vi "VIH Project Tree - Add Files - Build Item Tags.vi"(11 "Items Array":T2[](array[typedef])) -> (2 "Item Items Data":T1(array[cluster]), 3 "Item Parent Tags":string[](array[string]))   [LabVIEW 2014]
doc: "::: VI Helpeks :::\nCopyright (c) 2000-2026 Konstantin Shifershteyn. All rights reserved."
uses:
  _VIH HelpGen - Palette.llb/VIH HelpGen Typedef - Palette - Item Info Cluster.ctl
  _VIH HelpGen - Palette.llb/VIH HelpGen Typedef - Palette - Item Type Enum.ctl
  VIH Project Tree Typedef - Tree Item Type.ctl
panel:
  # "VI Helpeks\nCopyright (c) 2012-2026 Konstantin Shifershteyn"
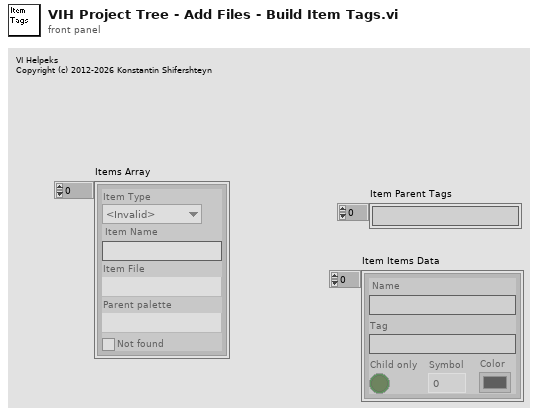
[diagram p1: front panel]
types:
  T1 = cluster{"Name":string, "Tag":string, "Child only":bool, "Symbol":i32, "Color":u32}[]
  T2 = typedef "VIH HelpGen Typedef - Palette - Item Info Cluster.ctl" = cluster{"Item Type":T3, "Item Name":string, "Item File":path, "Parent palette":path, "Not found":bool}
  T3 = typedef "VIH HelpGen Typedef - Palette - Item Type Enum.ctl" = enum32{"<Invalid>", "<unknown>", "VI", "Menu", "LV Func", "Express VI", "Poly VI", "CTL", "HTML"}
  T4 = cluster{"Name":string, "Tag":string, "Child only":bool, "Symbol":i32, "Color":u32}
  T5 = typedef "VIH Project Tree Typedef - Tree Item Type.ctl" = enum32{"<Invalid>", "Project", "Proj Files", "Proj Rules", "File Group", "Rule Group", "Any File", "LV Func", ".mnu", ".mnu (dyn)", ".vi", ".vi (dyn)", ".vit", ".vit (dyn)", ".ctl", ".ctl (dyn)", ".ctt", ".ctt (dyn)", "polyVI", "polyVI (dyn)", "expVI", "expVI (dyn)", "HTML", "PolyVI Inst"}
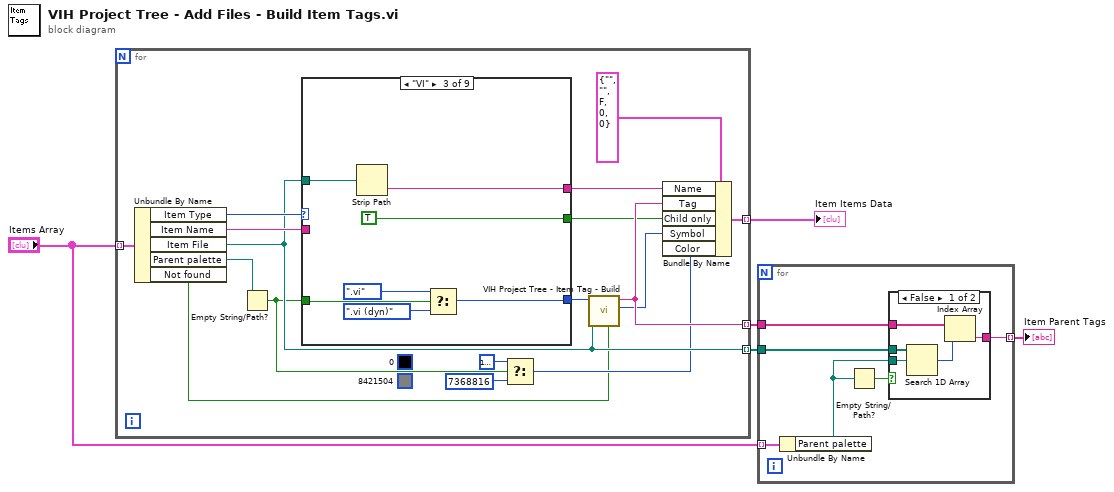
[diagram p0: block diagram]
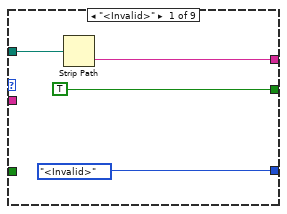
[diagram p3: hidden frame]
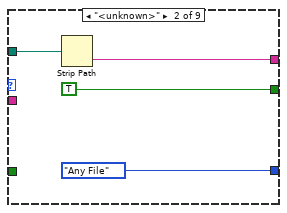
[diagram p4: hidden frame]
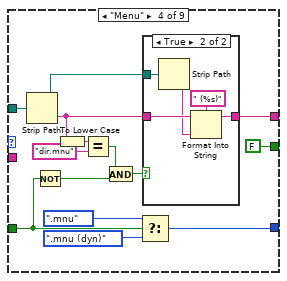
[diagram p5: hidden frame]
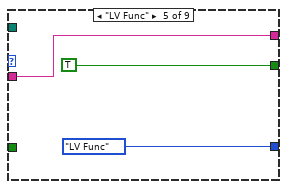
[diagram p7: hidden frame]
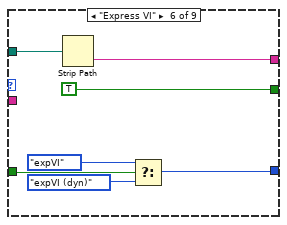
[diagram p8: hidden frame]
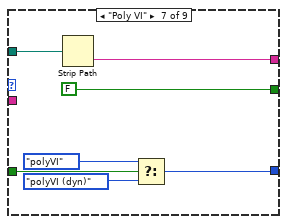
[diagram p9: hidden frame]
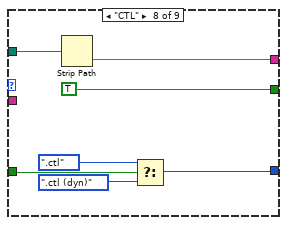
[diagram p10: hidden frame]
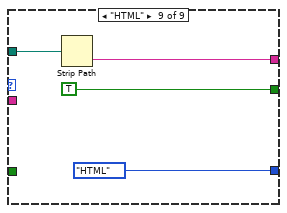
[diagram p11: hidden frame]
diagram:
  n1 = for {
    tunnel: "Items Array" -> [w22] mode=indexing
    tunnel: [w14] -> w3 mode=indexing
    tunnel: [w19] -> w4 mode=indexing
    tunnel: [w11] -> w1 mode=indexing
    (unwired) u32 8421504
    (unwired) u32 0
    n2 = Unbundle By Name(w22) -> ("Item Type"=w21:T3, "Item Name"=w20:string, "Item File"=w19:path, "Parent palette"=w18:path, "Not found"=w6:bool)
    n3 = Empty String/Path?(string/path=w18) -> (empty?=w10:bool)
    n4 = case shown="\"VI\"" w21 {
      tunnel: [TRUE TRUE TRUE FALSE TRUE TRUE FALSE TRUE TRUE] -> w12
      tunnel: w10 -> [_ _ w33 w44 _ w63 w70 w77 _]
      tunnel: [VIH_Project_Tree_Typedef_-_Tree_Item_Type."<Invalid>" ("Item Type") VIH_Project_Tree_Typedef_-_Tree_Item_Type."Any File" ("Item Type") w34 w48 VIH_Project_Tree_Typedef_-_Tree_Item_Type."LV Func" ("Item Type") w64 w71 w78 VIH_Project_Tree_Typedef_-_Tree_Item_Type."HTML" ("Item Type")] -> w17
      tunnel: w20 -> [_ _ _ _ w58 _ _ _ _]
      tunnel: [w23 w28 w31 w40 w58 w61 w68 w75 w83] -> w15
      tunnel: w19 -> [w24 w29 w32 w47 _ w62 w69 w76 w84]
      frame "<Invalid>" {
        n5 = Strip Path(path=w24) -> (name=w23:string)  [unwired: 1 out]
      }
      frame "<unknown>" {
        n6 = Strip Path(path=w29) -> (name=w28:string)  [unwired: 1 out]
      }
      frame "VI" {
        n7 = Strip Path(path=w32) -> (name=w31:string)  [unwired: 1 out]
        n8 = Select(t=VIH_Project_Tree_Typedef_-_Tree_Item_Type.".vi" ("Item Type"), s=w33, f=VIH_Project_Tree_Typedef_-_Tree_Item_Type.".vi (dyn)" ("Item Type")) -> (s? t:f=w34:T5)
      }
      frame "Menu" {
        n9 = Strip Path(path=w47) -> (stripped path=w38:path, name=w39:string)
        n10 = Not(x=w44) -> (.not. x?=w43:bool)
        n11 = To Lower Case(string=w39) -> (all lower case string=w46:string)
        n12 = Equal?(x=w46, y="dir.mnu") -> (x = y?=w42:bool)
        n13 = And(x=w42, y=w43) -> (x .and. y?=w41:bool)
        n14 = Select(t=VIH_Project_Tree_Typedef_-_Tree_Item_Type.".mnu" ("Item Type"), s=w44, f=VIH_Project_Tree_Typedef_-_Tree_Item_Type.".mnu (dyn)" ("Item Type")) -> (s? t:f=w48:T5)
        n15 = case shown="True" w41 {
          tunnel: [w52 w55] -> w40
          tunnel: w39 -> [w52 w56]
          tunnel: w38 -> [_ w57]
          frame False {
          }
          frame True {
            n16 = Strip Path(path=w57) -> (name=w54:string)  [unwired: 1 out]
            n17 = Format Into String(format string=" (%s)", initial string=w56, w54) -> (resulting string=w55:string)  [unwired: 1 in, 1 out]
          }
        }
      }
      frame "LV Func" {
      }
      frame "Express VI" {
        n18 = Strip Path(path=w62) -> (name=w61:string)  [unwired: 1 out]
        n19 = Select(t=VIH_Project_Tree_Typedef_-_Tree_Item_Type."expVI" ("Item Type"), s=w63, f=VIH_Project_Tree_Typedef_-_Tree_Item_Type."expVI (dyn)" ("Item Type")) -> (s? t:f=w64:T5)
      }
      frame "Poly VI" {
        n20 = Strip Path(path=w69) -> (name=w68:string)  [unwired: 1 out]
        n21 = Select(t=VIH_Project_Tree_Typedef_-_Tree_Item_Type."polyVI" ("Item Type"), s=w70, f=VIH_Project_Tree_Typedef_-_Tree_Item_Type."polyVI (dyn)" ("Item Type")) -> (s? t:f=w71:T5)
      }
      frame "CTL" {
        n22 = Strip Path(path=w76) -> (name=w75:string)  [unwired: 1 out]
        n23 = Select(t=VIH_Project_Tree_Typedef_-_Tree_Item_Type.".ctl" ("Item Type"), s=w77, f=VIH_Project_Tree_Typedef_-_Tree_Item_Type.".ctl (dyn)" ("Item Type")) -> (s? t:f=w78:T5)
      }
      frame "HTML" {
        n24 = Strip Path(path=w84) -> (name=w83:string)  [unwired: 1 out]
      }
    }
    n25 = Select(t=u32 16777228, s=w10, f=u32 7368816) -> (s? t:f=w8:u32)
    n26 = call "VIH Project Tree - Item Tag - Build.vi"("Not found"=w6, "Item File Path"=w19, "Item Type"=w17) -> ("Tree Item Symbol"=w13:i32, "Tree Item Tag"=w14:string)  [unwired: 7 in]
    n27 = Bundle By Name(cluster=T4 {"Name"="", "Tag"="", "Child only"=FALSE, "Symbol"=0, "Color"=0} ("Tree Item Data"), "Name"=w15, "Tag"=w14, "Child only"=w12, "Symbol"=w13, "Color"=w8) -> (w11:T4)
  }
  "Item Items Data" <- w1
  n28 = for {
    tunnel: "Items Array" -> [w91] mode=indexing
    tunnel: w4 -> [w90]
    tunnel: w3 -> [w89]
    tunnel: [w88] -> w2 mode=indexing
    n29 = Unbundle By Name(w91) -> ("Parent palette"=w87:path)
    n30 = Empty String/Path?(string/path=w87) -> (empty?=w86:bool)
    n31 = case shown="False" w86 {
      tunnel: w87 -> [w96 _]
      tunnel: w90 -> [w95 _]
      tunnel: w89 -> [w93 _]
      tunnel: [w92 _] -> w88
      frame False {
        n32 = Search 1D Array(1D array=w95, element=w96) -> (index of element=w94:i32)  [unwired: 1 in]
        n33 = Index Array(array=w93, index=w94) -> (element=w92:string)
      }
      frame True {
      }
    }
  }
  "Item Parent Tags" <- w2
